vi "Data_Read.vi"(8 "error in":errorcluster, 11 "reader ref in":refnum<k21>) -> (0 "error out":errorcluster, 2 "Array":i16[][](array[numeric]), 3 "reader ref out":refnum<k21>)   [LabVIEW 2025]
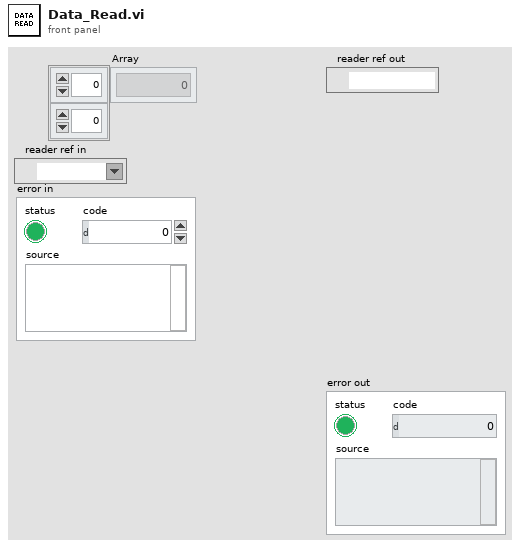
[diagram p1: front panel]
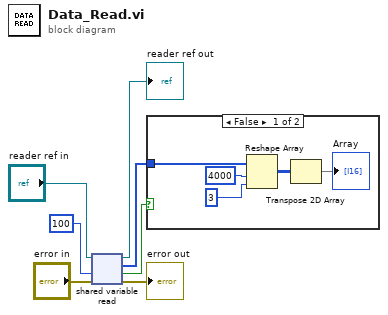
[diagram p0: block diagram]
diagram:
  n1 = shared-variable-read("reader ref in", "error in", 100 ("timeout ms (-1)")) -> (→"reader ref out":refnum<k21>, →"error out":errorcluster, w5:bool, w6:i16[])
  n2 = case shown="False" w5 {
    tunnel: w6 -> [w12 _]
    frame False {
      n3 = Reshape Array(w12, 4000 ("dimension size"), 3 ("dimension size")) -> (w9:i16[][])
      n4 = Transpose 2D Array(2D array=w9) -> (transposed array=→"Array":i16[][])
    }
    frame True {
    }
  }
